vi "Erase Metrics.vi"(8 "error in (no error)":errorcluster, 11 "Default Collector in":refnum<class "Default Collector.lvclass">) -> (0 "error out":errorcluster, 3 "Default Collector out":refnum<class "Default Collector.lvclass">)   [LabVIEW 2020, in "Collector.lvlib" / "Default Collector.lvclass"]
doc: "Deletes all the metrics owned by this collector."
uses:
  Default Collector.lvclass
  Default Collector.lvclass/Default Collector.ctl
  metrics/metric/Metric.lvclass
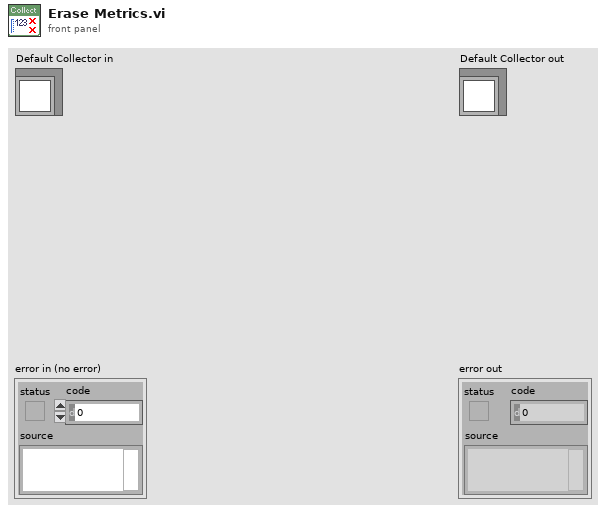
[diagram p1: front panel]
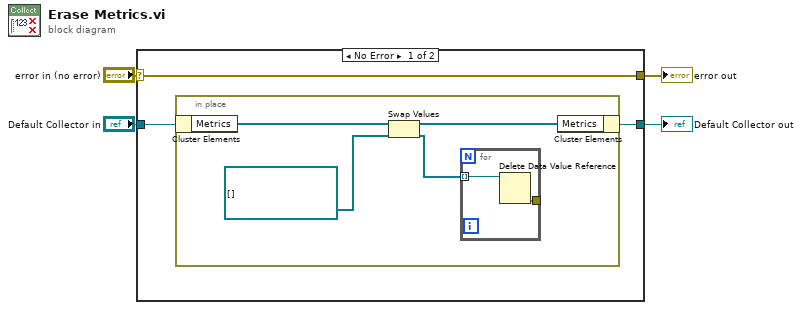
[diagram p0: block diagram]
diagram:
  n1 = case shown="No Error" "error in (no error)" {
    selector: "error in (no error)" -> [w7 w15]
    tunnel: [w7 w15] -> w3
    tunnel: [w5 w14] -> w1
    tunnel: "Default Collector in" -> [w6 w14]
    frame No Error {
      n2 = in-place {
        n3 = in-place-cluster #1(w6) -> ("Metrics"=w11:refnum<data-value>[])
        n4 = Swap Values(12:w11, 14:refnum<data-value>[] [] ("Metrics")) -> (1:w10:refnum<data-value>[], 3:w9:refnum<data-value>[])  [unwired: 1 in]
        n5 = for {
          tunnel: w9 -> [w12] mode=indexing
          tunnel: [w13] -> _
          n6 = Delete Data Value Reference(data value reference=w12) -> (error out=w13:errorcluster)  [unwired: 1 in, 1 out]
        }
        n7 = in-place-cluster #1("Metrics"=w10) -> (w5:refnum<class "Default Collector.lvclass">)
      }
    }
    frame Error {
    }
  }
  "error out" <- w3
  "Default Collector out" <- w1
